vi "Read Position.vi"(5 "Username":string, 6 "Password":string, 7 "Address":string, 8 "Error In":errorcluster) -> (0 "Error Out":errorcluster)   [LabVIEW 2018, in "Tests.lvlib" / "SFTP File.lvlib"]
uses:
  SFTP File.lvlib
  src/Toolkit/SFTP File/Type Definitions/Open Options.ctl
  src/Toolkit/SFTP File/SFTP File.lvclass/SFTP File.ctl
  src/Toolkit/SFTP/SFTP.lvclass/SFTP.ctl
  src/Toolkit/Session/Session.lvclass/Session.ctl
  src/Toolkit/SSH/SSH.lvclass/SSH.ctl
  src/Toolkit/SFTP/Utility/Read Shared Library.vi
  src/Toolkit/Session/Utility/Read Shared Library.vi
  src/Toolkit/SSH/Utility/Read Shared Library.vi
  src/Toolkit/SFTP File/Support/Open from SFTP.vi
  src/Toolkit/Support/Check Status.vi
  src/Toolkit/SFTP File/Support/Close to SFTP.vi
  <vilib>/addons/_JKI Toolkits/Caraya/classes/Test/Test.lvclass
  <vilib>/addons/_JKI Toolkits/Caraya/classes/Assert/Assert.lvclass
  src/Toolkit/SFTP File/SFTP File.lvclass
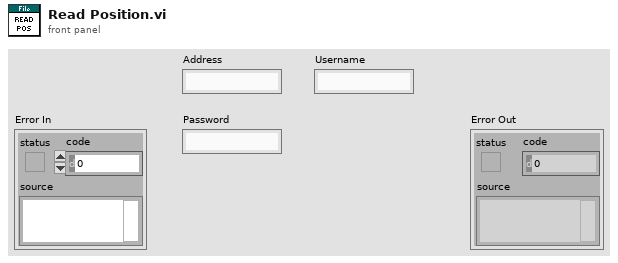
[diagram p1: front panel]
types:
  T1 = typedef "Toolkit.lvlib/SFTP File.lvclass/Open Options.ctl" = cluster{"Read":bool, "Write":bool, "Append":bool, "Create":bool, "Truncate":bool, "Exclude":bool}
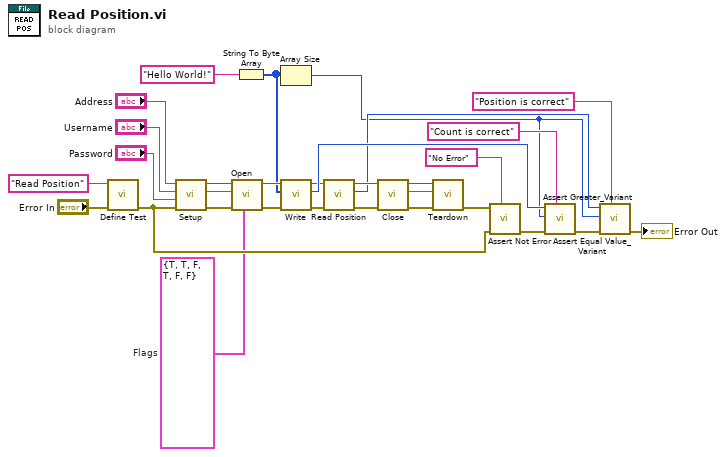
[diagram p0: block diagram]
diagram:
  w13 = T1 {"Read"=TRUE, "Write"=TRUE, "Append"=FALSE, "Create"=TRUE, "Truncate"=FALSE, "Exclude"=FALSE}  # Flags
  n1 = call <vilib>:"Define Test.vi"("error in (no error)"="Error In", "Label (VI Title)"="Read Position") -> ("error out"=w22:errorcluster)  [unwired: 9 in]
  n2 = call "Setup.vi"("Error In"=w22, "Password"="Password", "Username"="Username", "Address"="Address") -> ("Error Out"=w19:errorcluster, "Temporary File"=w1:string, "SFTP"=w20:refnum<class "SFTP.lvclass">)  [unwired: 5 in]
  n3 = call-poly "Open.vi"("Options"=w13, "Error In"=w19, "Remote Path"=w1, "SFTP"=w20) -> ("Error Out"=w16:errorcluster, "SFTP File"=w18:refnum<class "SFTP File.lvclass">)  [unwired: 6 in]
  n4 = String To Byte Array(string="Hello World!") -> (unsigned byte array=w14:u8[])
  n5 = Array Size(array=w14) -> (size(s)=w6:i32)
  n6 = call "Write.vi"("Error In"=w16, "Data"=w14, "SFTP File In"=w18) -> ("Error Out"=w9:errorcluster, "Count"=w17:i64, "SFTP File Out"=w12:refnum<class "SFTP File.lvclass">)  [unwired: 6 in]
  n7 = call "Read Position.vi"("Error In"=w9, "SFTP File In"=w12) -> ("Error Out"=w10:errorcluster, "Position"=w7:u64, "SFTP File Out"=w11:refnum<class "SFTP File.lvclass">)  [unwired: 7 in]
  n8 = call-poly "Close.vi"("Error In"=w10, "SFTP File"=w11) -> ("Error Out"=w3:errorcluster, "Remote Path"=w2:string, "SFTP"=w4:refnum<class "SFTP.lvclass">)  [unwired: 7 in]
  n9 = call "Teardown.vi"("Error In"=w3, "Temporary File"=w2, "SFTP"=w4) -> ("Error Out"=w21:errorcluster)  [unwired: 8 in]
  n10 = call <vilib>:"Assert Not Error.vi"("Label"="No Error", "error in (no error)"=w22, "Not Error?"=w21) -> ("error out"=w28:errorcluster)  [unwired: 8 in]
  n11 = call <vilib>:"Assert Greater_Variant.vi"("Label"="Count is correct", "error in (no error)"=w28, "Y"=w6, "X"=w17) -> ("error out"=w27:errorcluster)  [unwired: 7 in]
  n12 = call <vilib>:"Assert Equal Value_Variant.vi"("Label"="Position is correct", "error in (no error)"=w27, "Y"=w6, "X"=w7) -> ("error out"=→"Error Out":errorcluster)  [unwired: 7 in]
